vi "VIH Utility - MENU - Recent Paths Handler.vi"(6 "cmd (get list)":enum32{"get list", "delete", "insert"}(ring), 7 "max items (10)":i32=10, 8 "error in":errorcluster, 9 "Path":path, 10 "menu tag":string="RecentProjects", 11 "menubar":refnum<k9>) -> (0 "error out":errorcluster, 1 "item tags":string[](array[string]), 2 "dup menu tag":string, 3 "dup menubar":refnum<k9>)   [LabVIEW 2014]
doc: "::: VI Helpeks :::\nCopyright (c) 2000-2026 Konstantin Shifershteyn. All rights reserved."
panel:
  # "VI Helpeks\nCopyright (c) 2012-2026 Konstantin Shifershteyn"
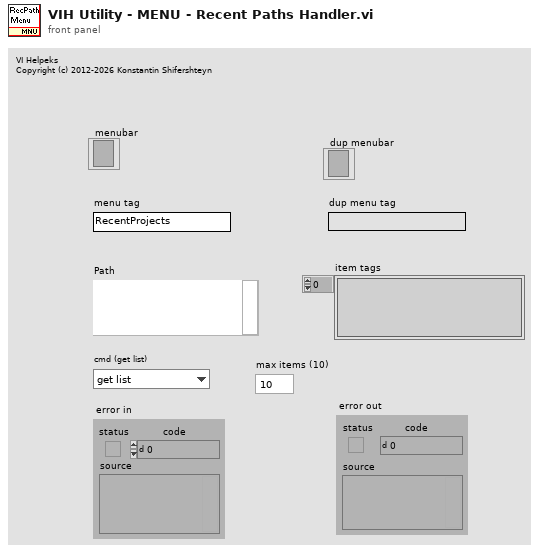
[diagram p1: front panel]
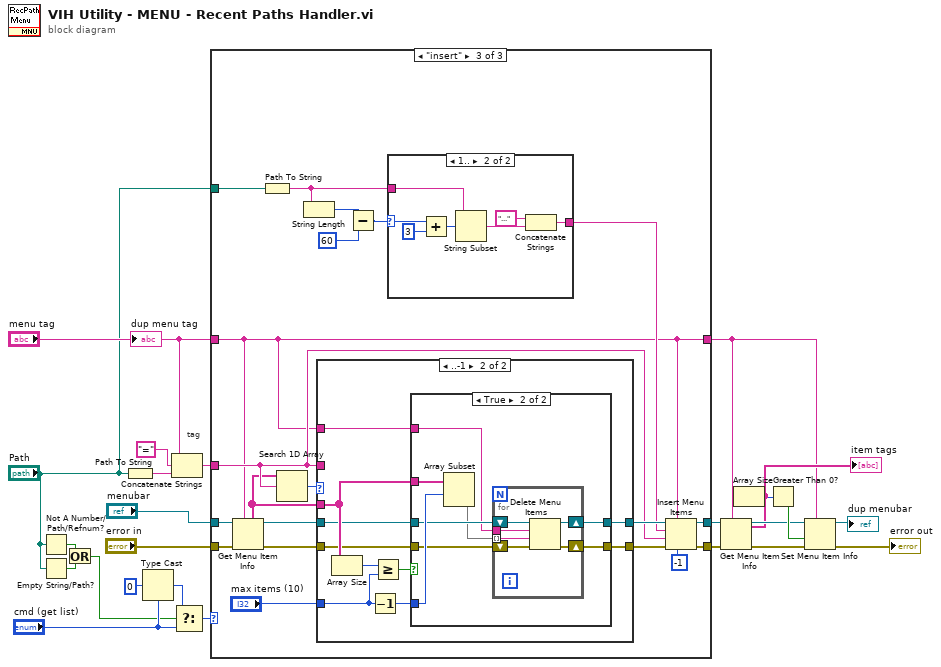
[diagram p0: block diagram]
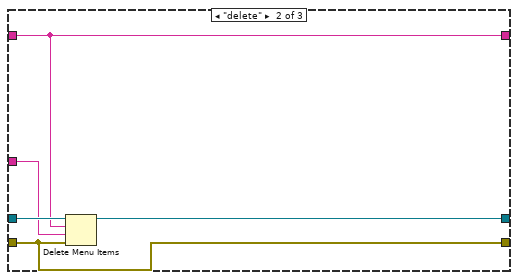
[diagram p3: hidden frame]
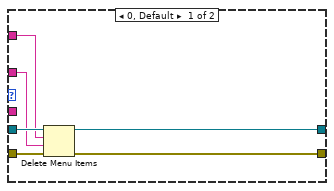
[diagram p5: hidden frame]
diagram:
  # "tag"
  n1 = Not A Number/Path/Refnum?(number/path/refnum="Path") -> (NaN/Path/Refnum?=w4:bool)
  n2 = Empty String/Path?(string/path="Path") -> (empty?=w3:bool)
  n3 = Or(x=w4, y=w3) -> (x .or. y?=w1:bool)
  n4 = Path To String(path="Path") -> (string=w22:string)
  n5 = Type Cast(type="cmd (get list)", x=0) -> (*(type *) &x=w10:enum32{"get list", "delete", "insert"})
  n6 = Concatenate Strings("menu tag", "=" ("string"), w22) -> (w23:string)
  n7 = Select(t=w10, s=w1, f="cmd (get list)") -> (s? t:f=w7:enum32{"get list", "delete", "insert"})
  n8 = case shown="\"insert\"" w7 {
    tunnel: "error in" -> [w27 w28 w42]
    tunnel: [w27 w28 w44] -> w18
    tunnel: "menubar" -> [w25 w32 w38]
    tunnel: "menu tag" -> [w26 w30 w39]
    tunnel: w23 -> [_ w31 w48]
    tunnel: "Path" -> [_ _ w37]
    tunnel: [w25 w29 w45] -> w19
    tunnel: [w26 w30 w39] -> w11
    frame "get list" {
    }
    frame "delete" {
      n9 = Delete Menu Items(6:w28, 7:w31, 8:w30, 9:w32) -> (3:w29:refnum<k9>)  [unwired: 1 out]
    }
    frame "insert" {
      n10 = Get Menu Item Info(7:w39, 8:w42, 11:w38) -> (0:w43:errorcluster, 3:w41:refnum<k9>, 5:w40:string[])  [unwired: 4 out]
      n11 = Path To String(path=w37) -> (string=w33:string)
      n12 = Search 1D Array(1D array=w40, element=w48) -> (index of element=w52:i32)  [unwired: 1 out]
      n13 = String Length(string=w33) -> (length=w36:i32)
      n14 = case shown="..-1" w52 {
        tunnel: w43 -> [w66 w72]
        tunnel: w41 -> [w65 w71]
        tunnel: w40 -> [_ w74]
        tunnel: w39 -> [w64 w70]
        tunnel: w48 -> [w63 _]
        tunnel: "max items (10)" -> [_ w73]
        tunnel: [w61 w69] -> w49
        tunnel: [w62 w68] -> w50
        frame 0, Default {
          n15 = Delete Menu Items(6:w66, 7:w63, 8:w64, 9:w65) -> (0:w62:errorcluster, 3:w61:refnum<k9>)
        }
        frame ..-1 {
          n16 = Array Size(array=w74) -> (size(s)=w76:i32)
          n17 = Decrement(x=w73) -> (x-1=w67:i32)
          n18 = Greater Or Equal?(x=w76, y=w73) -> (x >= y?=w75:bool)
          n19 = case shown="True" w75 {
            tunnel: w74 -> [_ w86]
            tunnel: w67 -> [_ w85]
            tunnel: w72 -> [w77 w84]
            tunnel: w71 -> [w78 w83]
            tunnel: w70 -> [_ w82]
            tunnel: [w77 w80] -> w68
            tunnel: [w78 w79] -> w69
            frame False {
            }
            frame True {
              n20 = Array Subset(array=w86, index=w85) -> (w81:string[])  [unwired: 1 in]
              n21 = for {
                shift-right: [w91] -> w79
                shift-left: w83 -> [w92]
                shift-right: [w89] -> w80
                shift-left: w84 -> [w90]
                tunnel: w82 -> [w88]
                tunnel: w81 -> [w87] mode=indexing
                n22 = Delete Menu Items(6:w90, 7:w87, 8:w88, 9:w92) -> (0:w89:errorcluster, 3:w91:refnum<k9>)
              }
            }
          }
        }
      }
      n23 = Subtract(x=w36, y=60) -> (x-y=w34:i32)
      n24 = case shown="1.." w34 {
        selector: w34 -> [_ w57]
        tunnel: w33 -> [w53 w58]
        tunnel: [w53 w56] -> w46
        frame ..0 {
        }
        frame 1.. {
          n25 = Add(x=w57, y=3) -> (x+y=w55:i32)
          n26 = String Subset(string=w58, offset (0)=w55) -> (substring=w60:string)  [unwired: 1 in]
          n27 = Concatenate Strings("..." ("string"), w60) -> (w56:string)
        }
      }
      n28 = Insert Menu Items(4:-1, 5:w39, 6:w50, 7:w48, 8:w46, 9:w49) -> (0:w44:errorcluster, 3:w45:refnum<k9>)  [unwired: 1 out]
    }
  }
  n29 = Get Menu Item Info(7:w11, 8:w18, 11:w19) -> (0:w15:errorcluster, 3:w16:refnum<k9>, 5:w14:string[])  [unwired: 4 out]
  "item tags" <- w14
  n30 = Array Size(array=w14) -> (size(s)=w20:i32)
  n31 = Greater Than 0?(x=w20) -> (x > 0?=w17:bool)
  n32 = Set Menu Item Info(7:w11, 8:w15, 9:w17, 11:w16) -> (0:→"error out":errorcluster, 3:→"dup menubar":refnum<k9>)  [unwired: 3 out]
  "dup menu tag" <- "menu tag"
